vi "Measure2.vi"() -> ()   [LabVIEW 2024]
uses:
  <vilib>/MakerHub/LINX/Public/Peripherals/Analog/Analog Read N Chans.vi
  <vilib>/MakerHub/LINX/Public/Peripherals/PWM/PWM Set Duty Cycle 1 Chan.vi
  <vilib>/MakerHub/LINX/Private/Local IO/LinxAnalogRead.vi
  <vilib>/MakerHub/LINX/Public/Utilities/Check Channel.vi
  <vilib>/MakerHub/LINX/Public/Utilities/Open Serial.vi
  Globals.vi
  <vilib>/MakerHub/LINX/Public/Peripherals/PWM/PWM Set Duty Cycle N Chans.vi
  <vilib>/addons/control/pid/pid.llb/PID (DBL).vi
  <vilib>/MakerHub/LINX/Private/Utilties/Generate Error.vi
  <vilib>/Utility/file.llb/Write Delimited Spreadsheet (string).vi
  <vilib>/MakerHub/LINX/LMH-LINX.lvlib
  <vilib>/addons/control/pid/NI_PID_pid.lvlib
  <vilib>/Analysis/NI_AALBase.lvlib
panel:
  out "Resistance Amplified":dbl
  out "Resistance A3":dbl
  in  "Current":dbl
  out "A2 (TH)":dbl
  out "A1 (Voltage)":dbl
  out "A0 (TC)":dbl
  out "Resistance Amplified":dbl(graph)
  out "A4":dbl
  out "A3":dbl
  out "Resistance A3":dbl(graph)
  out "TREF 2 Error":dbl
  out "TREF 2":dbl
  out "TREF 1 Error":dbl
  out "Seebeck Coeff":dbl
  out "TREF 1":dbl
  in  "Target TC":dbl format="%.2f"
  in  "Target TH":dbl format="%.2f"
  out "Auto":bool
  in  "Start Auto":bool
  in  "TH End":dbl(knob)=100.0 step=10.0 scale=0.0..100.0
  in  "TH Start":dbl(knob)=40.0 step=10.0 scale=0.0..100.0
  out "VOUT - 1.25":dbl(knob) scale=-1.0..1.0
  out "TC":dbl(slide) scale=0.0..100.0
  out "TH":dbl(slide) scale=0.0..100.0
  out "Voltage":dbl(graph)
  out "TH":dbl(graph)
  in  "Save to File":bool
  out "VOUT - 1.25":dbl
  out "TC":dbl(graph)
  out "TC":dbl
  in  "Stop Button":bool
  out "TH":dbl
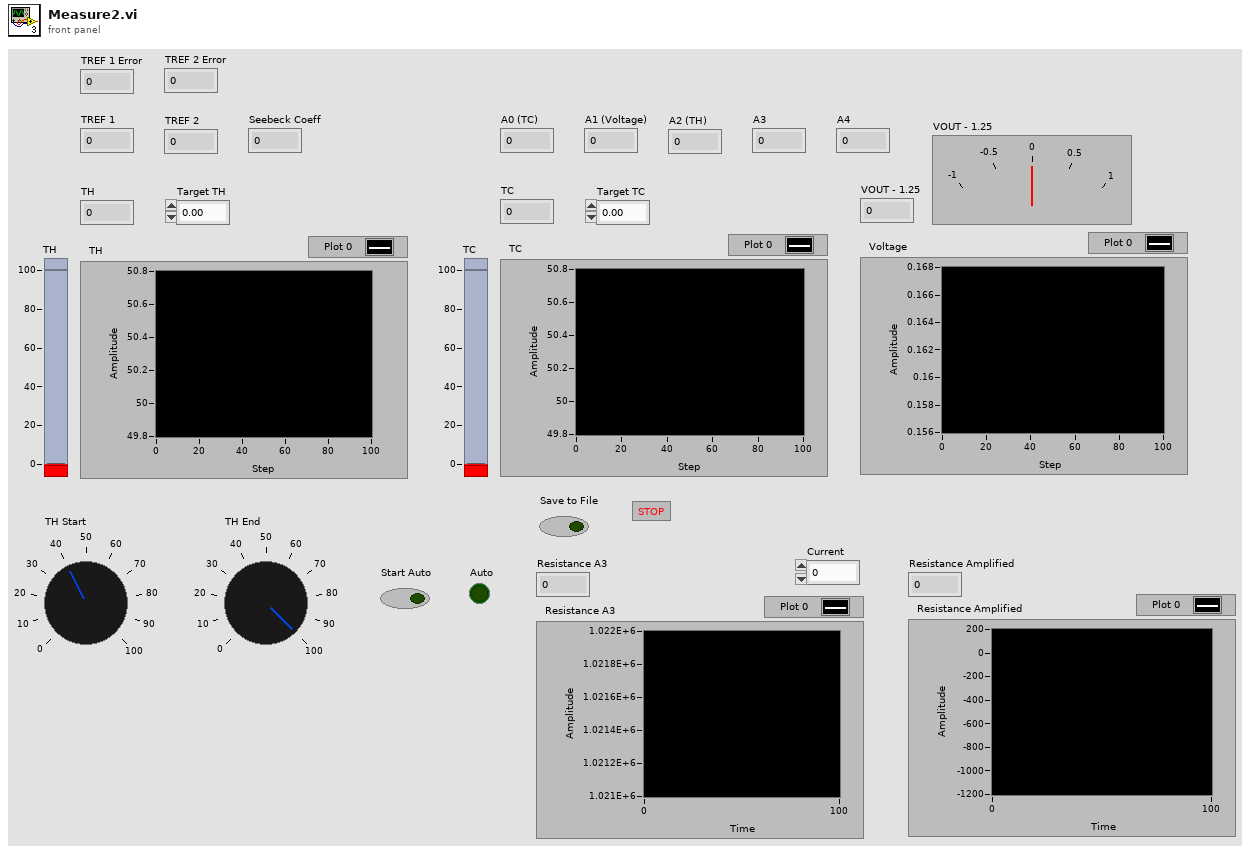
[diagram p1: front panel]
types:
  T1 = typedef "LMH-LINX.lvlib/LINX Ref.ctl" = cluster{"IO":T2, "Interface":T3, "LINX Device Config":T4}
  T2 = typedef "LMH-LINX.lvlib/Platform.ctl" = enum16{"Remote", "Local"}
  T3 = typedef "LMH-LINX.lvlib/Interface.ctl" = enum16{"Serial", "TCP"}
  T4 = typedef "LMH-LINX.lvlib/Device.lvlib/LINX Device Config.ctl" = cluster{"Interface":T3, "COM Port":refnum<visa-resource-name>, "TCP Configuration":T5, "Device Family":u8, "Device ID":u8, "Device Name":string, "TCP Ref":refnum<k5>, "Channels":T6}
  T5 = typedef "LMH-LINX.lvlib/Device.lvlib/TCP Config.ctl" = cluster{"IP Address":string, "Port":u16}
  T6 = typedef "LMH-LINX.lvlib/Channels.ctl" = cluster{"DI":u8[], "DO":u8[], "AI":u8[], "AO":u8[], "PWM":u8[], "QE":u8[], "UART":u8[], "I2C 2":u8[], "SPI":u8[], "CAN":u8[], "Servo":u8[], "AI Ref (V)":dbl, "AI Resolution (Bits)":u8, "AO Ref (V)":dbl, "AO Resolution (Bits)":u8}
  T7 = cluster{"proportional gain (Kc)":dbl, "integral time (Ti, min)":dbl, "derivative time (Td, min)":dbl}
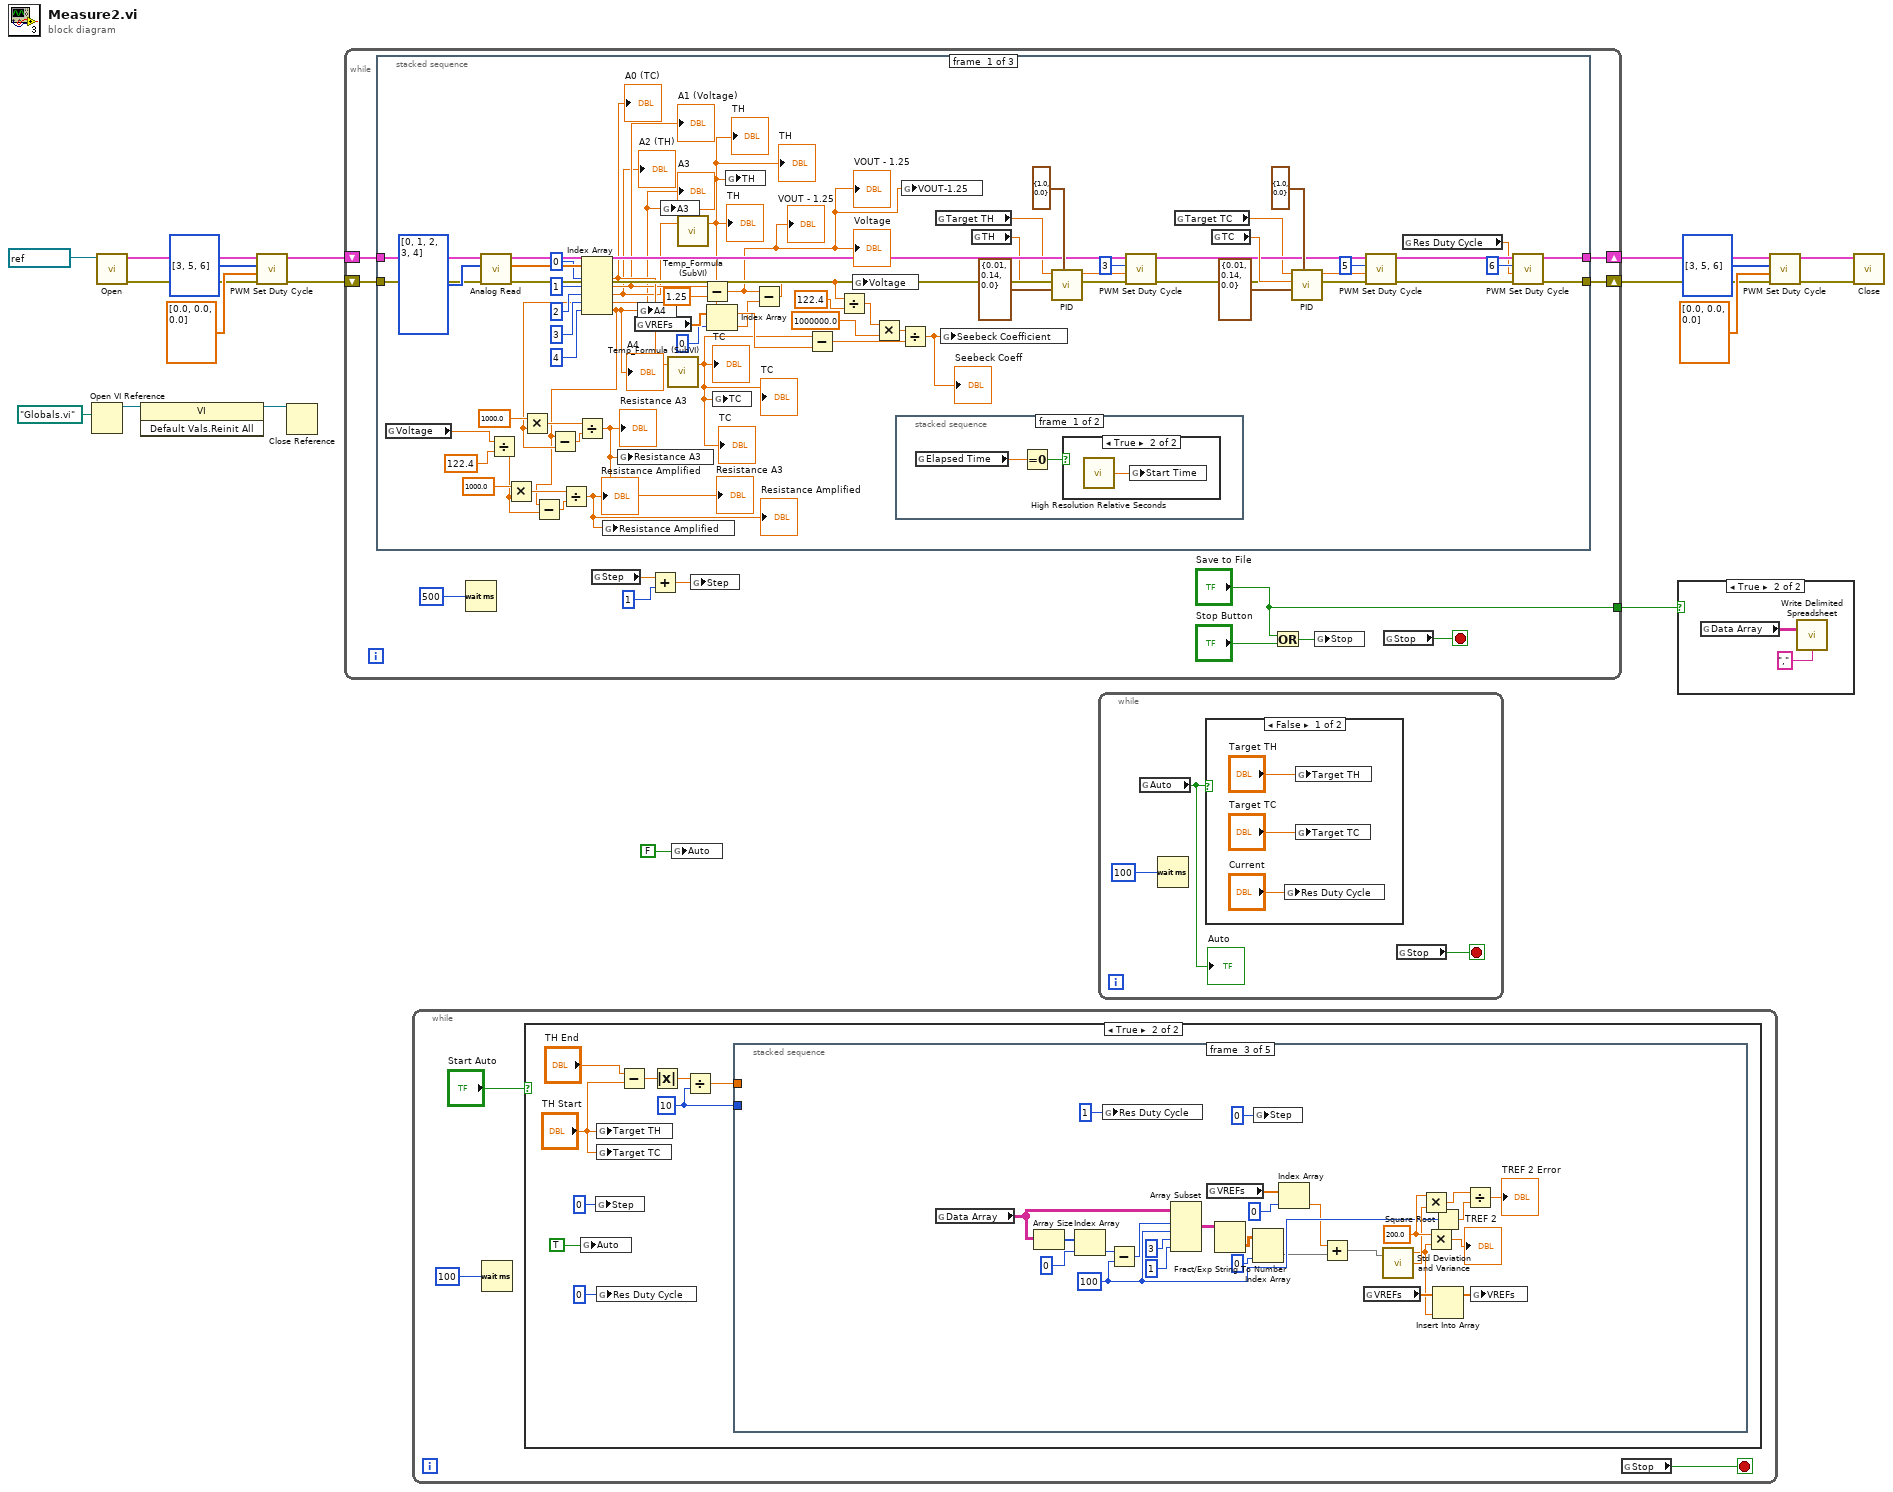
[diagram p0: block diagram]
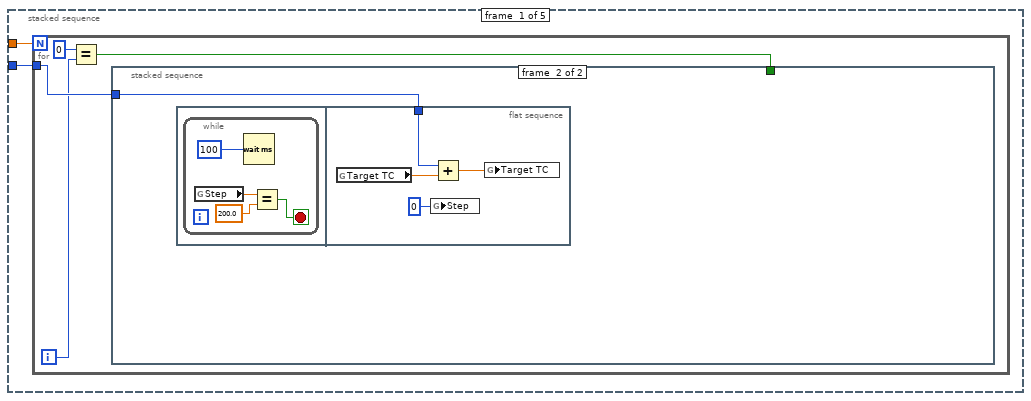
[diagram p3: hidden frame]
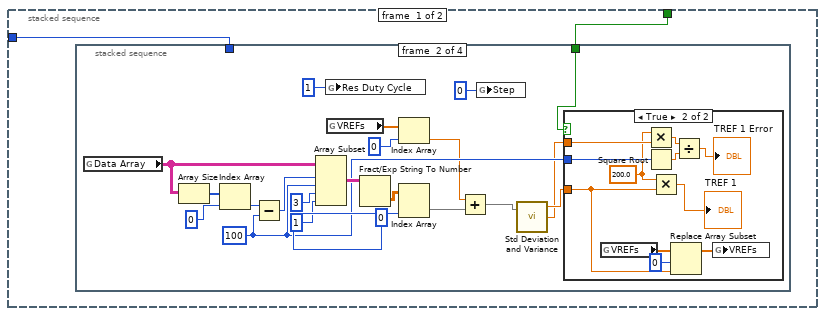
[diagram p4: hidden frame]
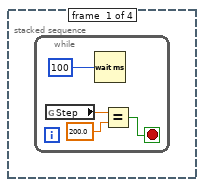
[diagram p5: hidden frame]
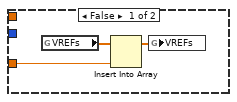
[diagram p6: hidden frame]
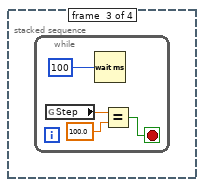
[diagram p7: hidden frame]
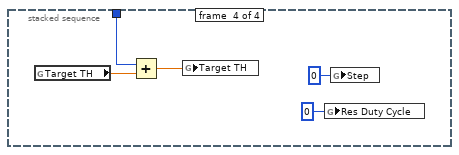
[diagram p8: hidden frame]
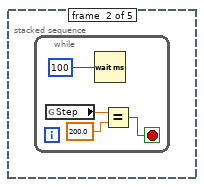
[diagram p9: hidden frame]
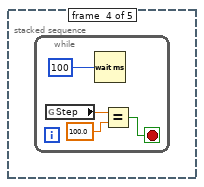
[diagram p10: hidden frame]
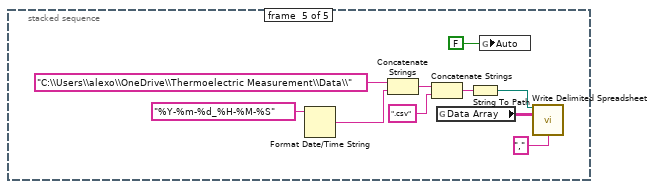
[diagram p11: hidden frame]
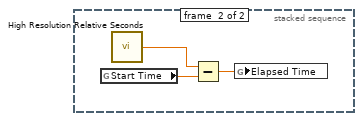
[diagram p15: hidden frame]
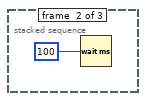
[diagram p16: hidden frame]
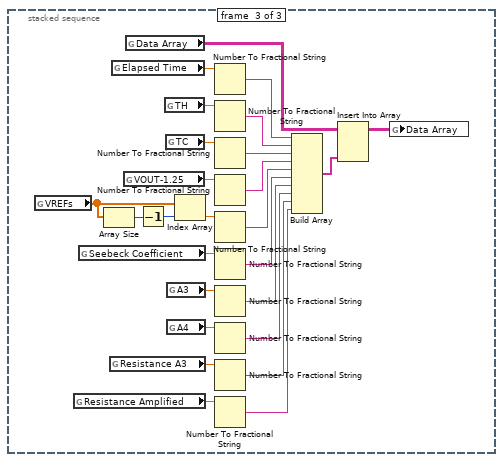
[diagram p17: hidden frame]
diagram:
  n1 = Open VI Reference(vi path=path "Globals.vi") -> (vi reference=w16:refnum<vi>)  [unwired: 5 in, 1 out]
  n2 = call-poly <vilib>:"Open.vi"("Serial Port"=refnum<visa-resource-name> "COM7") -> ("Error Out"=w8:errorcluster, "LINX Resource"=w11:T1)  [unwired: 8 in, 1 out]
  n3 = invoke class="VI" method="Default Vals.Reinit All"(reference=w16) -> (reference out=w15:refnum<vi>)  [unwired: 2 in, 2 out]
  n4 = call-poly <vilib>:"PWM Set Duty Cycle.vi"("Error In"=w8, "Duty Cycles"=dbl[] [0.0, 0.0, 0.0] ("Duty Cycle (0-1)"), "PWM Channels"=u8[] [3, 5, 6] ("PWM Channel"), "LINX Resource"=w11) -> ("Error Out"=w7:errorcluster, "LINX Resource"=w12:T1)  [unwired: 6 in]
  n5 = Close Reference(reference=w15) -> ()  [unwired: 1 in, 1 out]
  n6 = while {
    shift-right: [w29] -> w4
    shift-left: w12 -> [w30]
    shift-right: [w27] -> w1
    shift-left: w7 -> [w28]
    tunnel: ["Save to File"] -> w17
    stop <- w22 stop-if-true
    n7 = stacked-sequence {
      tunnel: w30 -> [w80 _ _]
      tunnel: [w41 _ _] -> w29
      tunnel: w28 -> [w79 _ _]
      tunnel: [w39 _ _] -> w27
      frame #0 {
        n8 = global read "Globals.vi" "Voltage"() -> (w36:dbl)
        n9 = call-poly <vilib>:"Analog Read.vi"("Error In"=w79, "AI Channel(s)"=i32[] [0, 1, 2, 3, 4], "LINX Resource"=w80) -> ("Error Out"=w77:errorcluster, "Voltages"=w88:dbl[], "LINX Resource"=w78:T1)  [unwired: 5 in, 1 out]
        n10 = Divide(x=w36, y=122.4) -> (x/y=w46:dbl)
        n11 = Multiply(x=1000.0 ("y"), y=w46) -> (x*y=w49:dbl)
        n12 = Index Array(array=w88, index #1=0 ("index"), index #2=1 ("index"), index #3=2 ("index"), index #4=3 ("index"), index #5=4 ("index")) -> (element #1=w45:dbl, element #2=w44:dbl, element #3=w43:dbl, element #4=w32:dbl, element #5=w31:dbl)
        "A3" <- w32
        "A4" <- w31
        "A0 (TC)" <- w45
        "A1 (Voltage)" <- w44
        "A2 (TH)" <- w43
        n13 = Multiply(x=1000.0 ("y"), y=w32) -> (x*y=w55:dbl)
        n14 = Subtract(x=w31, y=w46) -> (x-y=w47:dbl)
        n15 = Subtract(x=w31, y=w32) -> (x-y=w50:dbl)
        n16 = Divide(x=w49, y=w47) -> (x/y=w34:dbl)
        "Resistance Amplified" <- w34
        "Resistance Amplified" <- w34
        n17 = Divide(x=w55, y=w50) -> (x/y=w35:dbl)
        "Resistance A3" <- w35
        "Resistance A3" <- w35
        n18 = global write "Globals.vi" "Resistance Amplified"(w34) -> ()
        n19 = global write "Globals.vi" "Resistance A3"(w35) -> ()
        n20 = global read "Globals.vi" "VREFs"() -> (w59:dbl[])
        n21 = global write "Globals.vi" "A4"(w31) -> ()
        n22 = global write "Globals.vi" "A3"(w32) -> ()
        n23 = call "Temp_Formula (SubVI).vi"("In"=w45) -> ("Out"=w60:dbl)  [unwired: 1 in, 1 out]
        "TC" <- w60
        "TC" <- w60
        "TC" <- w60
        n24 = call "Temp_Formula (SubVI).vi"("In"=w43) -> ("Out"=w61:dbl)  [unwired: 1 in, 1 out]
        "TH" <- w61
        "TH" <- w61
        "TH" <- w61
        n25 = Subtract(x=w44, y=1.25) -> (x-y=w33:dbl)
        "VOUT - 1.25" <- w33
        "Voltage" <- w33
        "VOUT - 1.25" <- w33
        n26 = Index Array(array=w59, index=0) -> (element=w57:dbl)
        n27 = global write "Globals.vi" "TC"(w60) -> ()
        n28 = global write "Globals.vi" "TH"(w61) -> ()
        n29 = Subtract(x=w33, y=w57) -> (x-y=w56:dbl)
        n30 = Subtract(x=w60, y=w61) -> (x-y=w91:dbl)
        n31 = Divide(x=w56, y=122.4) -> (x/y=w62:dbl)
        n32 = global write "Globals.vi" "Voltage"(w56) -> ()
        n33 = Multiply(x=w62, y=1000000.0) -> (x*y=w65:dbl)
        n34 = stacked-sequence {
          frame #0 {
            n35 = global read "Globals.vi" "Elapsed Time"() -> (w92:dbl)
            n36 = Equal To 0?(x=w92) -> (x = 0?=w93:bool)
            n37 = case shown="True" w93 {
              frame False {
              }
              frame True {
                n38 = call <vilib>:"High Resolution Relative Seconds.vi"() -> ("relative seconds"=w94:dbl)
                n39 = global write "Globals.vi" "Start Time"(w94) -> ()
              }
            }
          }
          frame #1 {
            n40 = global read "Globals.vi" "Start Time"() -> (w95:dbl)
            n41 = call <vilib>:"High Resolution Relative Seconds.vi"() -> ("relative seconds"=w96:dbl)
            n42 = Subtract(x=w96, y=w95) -> (x-y=w97:dbl)
            n43 = global write "Globals.vi" "Elapsed Time"(w97) -> ()
          }
        }
        n44 = Divide(x=w65, y=w91) -> (x/y=w90:dbl)
        "Seebeck Coeff" <- w90
        n45 = global write "Globals.vi" "VOUT-1.25"(w33) -> ()
        n46 = global read "Globals.vi" "Target TH"() -> (w68:dbl)
        n47 = global write "Globals.vi" "Seebeck Coefficient"(w90) -> ()
        n48 = global read "Globals.vi" "TH"() -> (w76:dbl)
        n49 = call-poly <vilib>:"PID.vi"("output range"=cluster{"output high":dbl, "output low":dbl} {"output high"=1.0, "output low"=0.0}, "PID gains"=T7 {"proportional gain (Kc)"=0.01, "integral time (Ti, min)"=0.14, "derivative time (Td, min)"=0.0}, "process variable"=w76, "setpoint"=w68) -> ("output"=w84:dbl)  [unwired: 6 in, 1 out]
        n50 = call-poly <vilib>:"PWM Set Duty Cycle.vi"("Error In"=w77, "Duty Cycle (0-1)"=w84, "PWM Channel"=u8 3, "LINX Resource"=w78) -> ("Error Out"=w69:errorcluster, "LINX Resource"=w70:T1)  [unwired: 6 in]
        n51 = global read "Globals.vi" "Target TC"() -> (w67:dbl)
        n52 = global read "Globals.vi" "TC"() -> (w71:dbl)
        n53 = call-poly <vilib>:"PID.vi"("output range"=cluster{"output high":dbl, "output low":dbl} {"output high"=1.0, "output low"=0.0}, "PID gains"=T7 {"proportional gain (Kc)"=0.01, "integral time (Ti, min)"=0.14, "derivative time (Td, min)"=0.0}, "process variable"=w71, "setpoint"=w67) -> ("output"=w75:dbl)  [unwired: 6 in, 1 out]
        n54 = call-poly <vilib>:"PWM Set Duty Cycle.vi"("Error In"=w69, "Duty Cycle (0-1)"=w75, "PWM Channel"=u8 5, "LINX Resource"=w70) -> ("Error Out"=w40:errorcluster, "LINX Resource"=w42:T1)  [unwired: 6 in]
        n55 = global read "Globals.vi" "Res Duty Cycle"() -> (w37:dbl)
        n56 = call-poly <vilib>:"PWM Set Duty Cycle.vi"("Error In"=w40, "Duty Cycle (0-1)"=w37, "PWM Channel"=u8 6, "LINX Resource"=w42) -> ("Error Out"=w39:errorcluster, "LINX Resource"=w41:T1)  [unwired: 6 in]
      }
      frame #1 {
        n57 = Wait (ms)(milliseconds to wait=u32 100) -> ()  [unwired: 1 out]
      }
      frame #2 {
        n58 = global read "Globals.vi" "VREFs"() -> (w111:dbl[])
        n59 = global read "Globals.vi" "Resistance Amplified"() -> (w102:dbl)
        n60 = global read "Globals.vi" "Seebeck Coefficient"() -> (w115:dbl)
        n61 = Array Size(array=w111) -> (size(s)=w110:i32)
        n62 = global read "Globals.vi" "Resistance A3"() -> (w101:dbl)
        n63 = global read "Globals.vi" "Elapsed Time"() -> (w113:dbl)
        n64 = global read "Globals.vi" "VOUT-1.25"() -> (w120:dbl)
        n65 = global read "Globals.vi" "Data Array"() -> (w123:string[][])
        n66 = Decrement(x=w110) -> (x-1=w109:i32)
        n67 = global read "Globals.vi" "TH"() -> (w116:dbl)
        n68 = global read "Globals.vi" "TC"() -> (w118:dbl)
        n69 = global read "Globals.vi" "A3"() -> (w103:dbl)
        n70 = global read "Globals.vi" "A4"() -> (w104:dbl)
        n71 = Index Array(array=w111, index=w109) -> (element=w108:dbl)
        n72 = Number To Fractional String(number=w113) -> (F-format string=w114:string)  [unwired: 3 in]
        n73 = Number To Fractional String(number=w116) -> (F-format string=w117:string)  [unwired: 3 in]
        n74 = Number To Fractional String(number=w118) -> (F-format string=w119:string)  [unwired: 3 in]
        n75 = Number To Fractional String(number=w120) -> (F-format string=w121:string)  [unwired: 3 in]
        n76 = Number To Fractional String(number=w108) -> (F-format string=w107:string)  [unwired: 3 in]
        n77 = Number To Fractional String(number=w115) -> (F-format string=w112:string)  [unwired: 3 in]
        n78 = Number To Fractional String(number=w103) -> (F-format string=w106:string)  [unwired: 3 in]
        n79 = Number To Fractional String(number=w104) -> (F-format string=w105:string)  [unwired: 3 in]
        n80 = Number To Fractional String(number=w101) -> (F-format string=w100:string)  [unwired: 3 in]
        n81 = Number To Fractional String(number=w102) -> (F-format string=w99:string)  [unwired: 3 in]
        n82 = Build Array(w114, w117, w119, w121, w107, w112, w106, w105, w100, w99) -> (w122:string[])
        n83 = Insert Into Array(array=w123, new element=w122) -> (w124:string[][])  [unwired: 2 in]
        n84 = global write "Globals.vi" "Data Array"(w124) -> ()
      }
    }
    n85 = Wait (ms)(milliseconds to wait=u32 500) -> ()  [unwired: 1 out]
    n86 = global read "Globals.vi" "Step"() -> (w21:dbl)
    n87 = Add(x=w21, y=1) -> (x+y=w20:dbl)
    n88 = global write "Globals.vi" "Step"(w20) -> ()
    n89 = Or(x="Save to File", y="Stop Button") -> (x .or. y?=w23:bool)
    n90 = global write "Globals.vi" "Stop"(w23) -> ()
    n91 = global read "Globals.vi" "Stop"() -> (w22:bool)
  }
  n92 = while {
    stop <- w126 stop-if-true
    n93 = Wait (ms)(milliseconds to wait=u32 100) -> ()  [unwired: 1 out]
    n94 = case shown="True" "Start Auto" {
      frame False {
      }
      frame True {
        w131 = 10
        n95 = global write "Globals.vi" "Auto"(TRUE) -> ()
        n96 = global write "Globals.vi" "Step"(0) -> ()
        n97 = global write "Globals.vi" "Target TH"("TH Start") -> ()
        n98 = global write "Globals.vi" "Target TC"("TH Start") -> ()
        n99 = global write "Globals.vi" "Res Duty Cycle"(0) -> ()
        n100 = Subtract(x="TH End", y="TH Start") -> (x-y=w134:dbl)
        n101 = Absolute Value(x=w134) -> (abs(x)=w133:dbl)
        n102 = Divide(x=w133, y=w131) -> (x/y=w130:dbl)
        n103 = stacked-sequence {
          tunnel: w130 -> [w138 _ _ _ _]
          tunnel: w131 -> [w137 _ _ _ _]
          frame #0 {
            n104 = for {
              N: w138 -> [_]
              tunnel: w137 -> [w142]
              i -> [w139]
              n105 = Equal?(x=0 ("y"), y=w139) -> (x = y?=w141:bool)
              n106 = stacked-sequence {
                tunnel: w142 -> [w144 w193]
                tunnel: w141 -> [w143 _]
                frame #0 {
                  n107 = stacked-sequence {
                    tunnel: w144 -> [_ _ _ w190]
                    tunnel: w143 -> [_ w169 _ _]
                    frame #0 {
                      n108 = while {
                        stop <- w145 stop-if-true
                        n109 = global read "Globals.vi" "Step"() -> (w147:dbl)
                        n110 = Wait (ms)(milliseconds to wait=u32 100) -> ()  [unwired: 1 out]
                        n111 = Equal?(x=w147, y=200.0) -> (x = y?=w145:bool)
                      }
                    }
                    frame #1 {
                      w157 = 100 ("y")
                      n112 = global read "Globals.vi" "Data Array"() -> (w163:string[][])
                      n113 = Array Size(array=w163) -> (size(s)=w164:i32[])
                      n114 = Index Array(array=w164, index=0) -> (element=w165:i32)
                      n115 = Subtract(x=w165, y=w157) -> (x-y=w166:i32)
                      n116 = Array Subset(array=w163, index (row)=w166, length (row)=w157, index (col)=3 ("index"), length (col)=1 ("length")) -> (w167:string[][])
                      n117 = global write "Globals.vi" "Res Duty Cycle"(1) -> ()
                      n118 = global read "Globals.vi" "VREFs"() -> (w155:dbl[])
                      n119 = Fract/Exp String To Number(string=w167) -> (number=w168:dbl[][])  [unwired: 3 in, 1 out]
                      n120 = Index Array(array=w155, index=0) -> (element=w153:dbl)
                      n121 = Index Array(array=w168, index (col)=0 ("dimension size")) -> (element=w151:dbl[])  [unwired: 1 in]
                      n122 = Add(x=w153, y=w151) -> (x+y=w152:dbl[])
                      n123 = global write "Globals.vi" "Step"(0) -> ()
                      n124 = call <vilib>:"Std Deviation and Variance.vi"("X"=w152) -> ("mean"=w158:dbl, "standard deviation"=w156:dbl)  [unwired: 1 in, 1 out]
                      n125 = case shown="True" w169 {
                        tunnel: w158 -> [w170 w174]
                        tunnel: w157 -> [_ w181]
                        tunnel: w156 -> [_ w180]
                        frame False {
                          n126 = global read "Globals.vi" "VREFs"() -> (w171:dbl[])
                          n127 = Insert Into Array(array=w171, new element=w170) -> (w172:dbl[])  [unwired: 1 in]
                          n128 = global write "Globals.vi" "VREFs"(w172) -> ()
                        }
                        frame True {
                          w177 = 200.0 ("x")
                          n129 = global read "Globals.vi" "VREFs"() -> (w176:dbl[])
                          n130 = Multiply(x=w177, y=w180) -> (x*y=w182:dbl)
                          n131 = Square Root(x=w181) -> (sqrt(x)=w178:dbl)
                          n132 = Multiply(x=w177, y=w174) -> (x*y=→"TREF 1":dbl)
                          n133 = Replace Array Subset(array=w176, new element=w174, index=0) -> (w175:dbl[])
                          n134 = Divide(x=w182, y=w178) -> (x/y=→"TREF 1 Error":dbl)
                          n135 = global write "Globals.vi" "VREFs"(w175) -> ()
                        }
                      }
                    }
                    frame #2 {
                      n136 = while {
                        stop <- w184 stop-if-true
                        n137 = global read "Globals.vi" "Step"() -> (w186:dbl)
                        n138 = Wait (ms)(milliseconds to wait=u32 100) -> ()  [unwired: 1 out]
                        n139 = Equal?(x=w186, y=100.0) -> (x = y?=w184:bool)
                      }
                    }
                    frame #3 {
                      n140 = global read "Globals.vi" "Target TH"() -> (w192:dbl)
                      n141 = Add(x=w190, y=w192) -> (x+y=w191:dbl)
                      n142 = global write "Globals.vi" "Target TH"(w191) -> ()
                      n143 = global write "Globals.vi" "Res Duty Cycle"(0) -> ()
                      n144 = global write "Globals.vi" "Step"(0) -> ()
                    }
                  }
                }
                frame #1 {
                  n145 = flat-sequence {
                    tunnel: w193 -> [w199]
                    frame #0 {
                      n146 = while {
                        stop <- w194 stop-if-true
                        n147 = global read "Globals.vi" "Step"() -> (w196:dbl)
                        n148 = Wait (ms)(milliseconds to wait=u32 100) -> ()  [unwired: 1 out]
                        n149 = Equal?(x=w196, y=200.0) -> (x = y?=w194:bool)
                      }
                    }
                    frame #1 {
                      n150 = global read "Globals.vi" "Target TC"() -> (w200:dbl)
                      n151 = global write "Globals.vi" "Step"(0) -> ()
                      n152 = Add(x=w199, y=w200) -> (x+y=w201:dbl)
                      n153 = global write "Globals.vi" "Target TC"(w201) -> ()
                    }
                  }
                }
              }
            }
          }
          frame #1 {
            n154 = while {
              stop <- w202 stop-if-true
              n155 = global read "Globals.vi" "Step"() -> (w204:dbl)
              n156 = Wait (ms)(milliseconds to wait=u32 100) -> ()  [unwired: 1 out]
              n157 = Equal?(x=w204, y=200.0) -> (x = y?=w202:bool)
            }
          }
          frame #2 {
            w223 = 200.0 ("x")
            w218 = 100 ("y")
            n158 = global read "Globals.vi" "Data Array"() -> (w232:string[][])
            n159 = Array Size(array=w232) -> (size(s)=w230:i32[])
            n160 = Index Array(array=w230, index=0) -> (element=w228:i32)
            n161 = global write "Globals.vi" "Res Duty Cycle"(1) -> ()
            n162 = Subtract(x=w228, y=w218) -> (x-y=w227:i32)
            n163 = Array Subset(array=w232, index (row)=w227, length (row)=w218, index (col)=3 ("index"), length (col)=1 ("length")) -> (w224:string[][])
            n164 = global read "Globals.vi" "VREFs"() -> (w212:dbl[])
            n165 = Fract/Exp String To Number(string=w224) -> (number=w217:dbl[][])  [unwired: 3 in, 1 out]
            n166 = Index Array(array=w217, index (col)=0 ("dimension size")) -> (element=w208:dbl[])  [unwired: 1 in]
            n167 = global write "Globals.vi" "Step"(0) -> ()
            n168 = Index Array(array=w212, index=0) -> (element=w210:dbl)
            n169 = Add(x=w210, y=w208) -> (x+y=w209:dbl[])
            n170 = global read "Globals.vi" "VREFs"() -> (w214:dbl[])
            n171 = call <vilib>:"Std Deviation and Variance.vi"("X"=w209) -> ("mean"=w213:dbl, "standard deviation"=w222:dbl)  [unwired: 1 in, 1 out]
            n172 = Multiply(x=w223, y=w222) -> (x*y=w221:dbl)
            n173 = Multiply(x=w223, y=w213) -> (x*y=→"TREF 2":dbl)
            n174 = Square Root(x=w218) -> (sqrt(x)=w220:dbl)
            n175 = Insert Into Array(array=w214, new element=w213) -> (w215:dbl[])  [unwired: 1 in]
            n176 = Divide(x=w221, y=w220) -> (x/y=→"TREF 2 Error":dbl)
            n177 = global write "Globals.vi" "VREFs"(w215) -> ()
          }
          frame #3 {
            n178 = while {
              stop <- w233 stop-if-true
              n179 = global read "Globals.vi" "Step"() -> (w235:dbl)
              n180 = Wait (ms)(milliseconds to wait=u32 100) -> ()  [unwired: 1 out]
              n181 = Equal?(x=w235, y=100.0) -> (x = y?=w233:bool)
            }
          }
          frame #4 {
            n182 = Format Date/Time String(time format string (%c)="%Y-%m-%d_%H-%M-%S") -> (date/time string=w241:string)  [unwired: 2 in]
            n183 = Concatenate Strings("C:\\Users\\alexo\\OneDrive\\Thermoelectric Measurement\\Data\\" ("string"), w241) -> (w242:string)
            n184 = Concatenate Strings(w242, ".csv" ("string")) -> (w239:string)
            n185 = global read "Globals.vi" "Data Array"() -> (w245:string[][])
            n186 = String To Path(string=w239) -> (path=w238:path)
            n187 = global write "Globals.vi" "Auto"(FALSE) -> ()
            n188 = call-poly <vilib>:"Write Delimited Spreadsheet.vi"("file path (dialog if empty)"=w238, "2D data"=w245, "delimiter (\\t)"="," ("delimiter (\\t)")) -> ()  [unwired: 11 in, 2 out]
          }
        }
      }
    }
    n189 = global read "Globals.vi" "Stop"() -> (w126:bool)
  }
  n190 = global write "Globals.vi" "Auto"(FALSE) -> ()
  n191 = while {
    stop <- w248 stop-if-true
    n192 = global read "Globals.vi" "Auto"() -> (w249:bool)
    "Auto" <- w249
    n193 = Wait (ms)(milliseconds to wait=u32 100) -> ()  [unwired: 1 out]
    n194 = case shown="False" w249 {
      frame False {
        n195 = global write "Globals.vi" "Res Duty Cycle"("Current") -> ()
        n196 = global write "Globals.vi" "Target TH"("Target TH") -> ()
        n197 = global write "Globals.vi" "Target TC"("Target TC") -> ()
      }
      frame True {
      }
    }
    n198 = global read "Globals.vi" "Stop"() -> (w248:bool)
  }
  n199 = case shown="True" w17 {
    frame False {
    }
    frame True {
      n200 = global read "Globals.vi" "Data Array"() -> (w254:string[][])
      n201 = call-poly <vilib>:"Write Delimited Spreadsheet.vi"("2D data"=w254, "delimiter (\\t)"="," ("delimiter (\\t)")) -> ()  [unwired: 12 in, 2 out]
    }
  }
  n202 = call-poly <vilib>:"PWM Set Duty Cycle.vi"("Error In"=w1, "Duty Cycles"=dbl[] [0.0, 0.0, 0.0] ("Duty Cycle (0-1)"), "PWM Channels"=u8[] [3, 5, 6] ("PWM Channel"), "LINX Resource"=w4) -> ("Error Out"=w2:errorcluster, "LINX Resource"=w3:T1)  [unwired: 6 in]
  n203 = call <vilib>:"Close.vi"("Error In"=w2, "LINX Resource"=w3) -> ()  [unwired: 9 in, 1 out]
